vi "Run Panel VI.vi"(8 "error in (no error)":errorcluster, 11 "Panel in":refnum<class "Panel.lvclass">) -> (0 "error out":errorcluster, 3 "Panel out":refnum<class "Panel.lvclass">)   [LabVIEW 2020, in "OOPanel.lvlib" / "Panel.lvclass"]
uses:
  Panel.lvclass
  Panel.lvclass/Panel.ctl
  Visibility State.ctl
  <vilib>/Utility/error.llb/Error Cluster From Error Code.vi
  <vilib>/ErrorRing/Error Ring.xnode
  OOPanel.lvlib
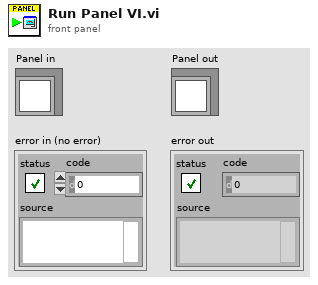
[diagram p1: front panel]
types:
  T1 = typedef "OOPanel.lvlib/Visibility State.ctl" = enum16{"Idle", "Closed", "Hidden", "Visible", "Subpanel", "Hidden Subpanel"}
  T2 = enum32{"invalid scope", "public", "private", "protected", "community"}
  T3 = enum32{"Invalid", "Standard", "Closed", "Hidden", "Minimized", "Maximized"}
  T4 = typedef "OOPanel.lvlib/Panel.lvclass/Ref Data.ctl" = cluster{"Panel Ref":refnum<vi>, "SubPanel":refnum<vi>, "Close":bool, "Running":bool, "State":T1}
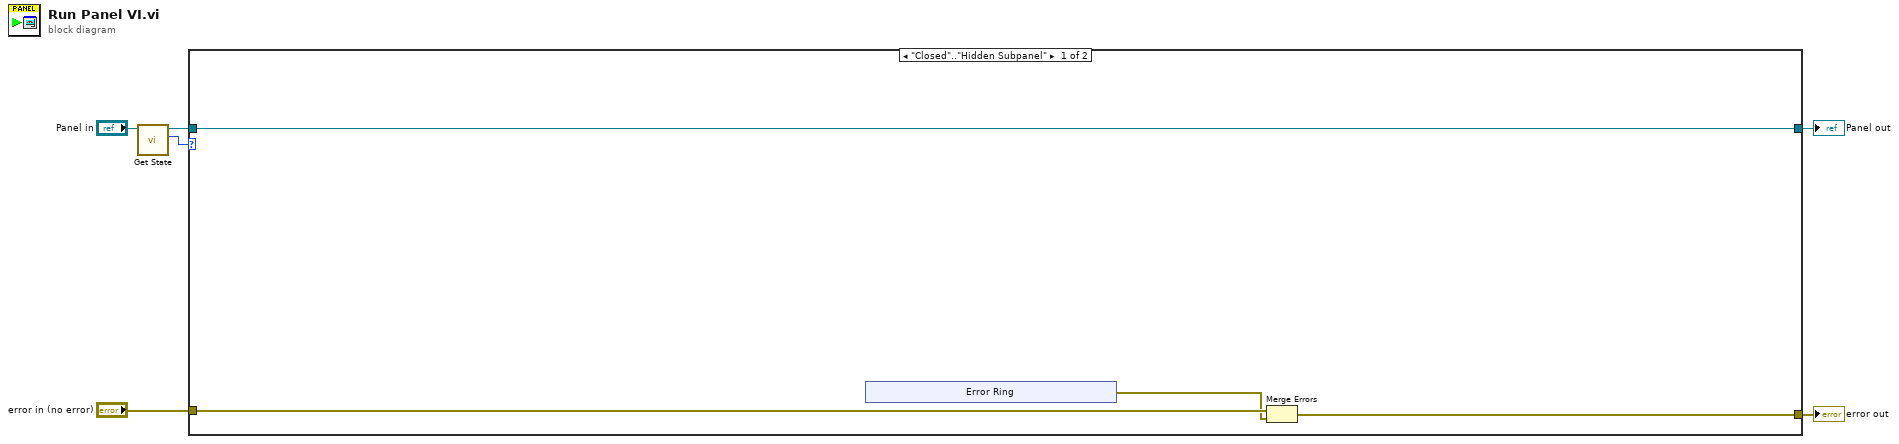
[diagram p0: block diagram]
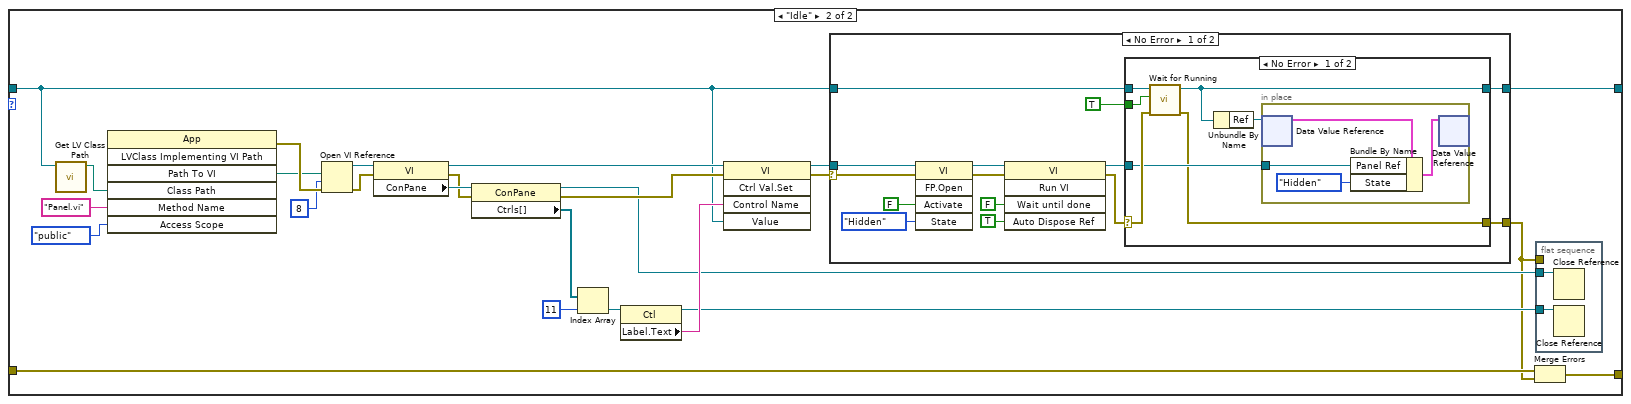
[diagram p2: hidden frame]
diagram:
  n1 = call "Get State.vi"("Panel in"="Panel in") -> ("State"=w1:T1, "Panel out"=w2:refnum<class "Panel.lvclass">)  [unwired: 8 in, 1 out]
  n2 = case shown="\"Closed\"..\"Hidden Subpanel\"" w1 {
    tunnel: "error in (no error)" -> [w9 w38]
    tunnel: [w10 w24] -> w5
    tunnel: [w7 w23] -> w4
    tunnel: w2 -> [w10 w18]
    frame "Closed".."Hidden Subpanel" {
      n3 = xnode "Error Ring"() -> ("error out"=w8:errorcluster)
      n4 = Merge Errors(w9, w8) -> (w7:errorcluster)
    }
    frame "Idle" {
      n5 = call <vilib>:"Get LV Class Path.vi"("object"=w18) -> ("class path"=w17:path)  [unwired: 9 in, 1 out]
      n6 = invoke class="App" method="LVClass Implementing VI Path"("Class Path"=w17, "Method Name"="Panel.vi", "Access Scope"=T2."public") -> (error out=w39:errorcluster, "Path To VI"=w16:path)  [unwired: 4 in, 5 out]
      n7 = Open VI Reference(vi path=w16, options=8, error in (no error)=w39) -> (vi reference=w37:refnum<vi>, error out=w36:errorcluster)  [unwired: 3 in]
      n8 = property class="VI"(reference=w37, error in=w36) -> (reference out=w32:refnum<vi>, error out=w30:errorcluster, "ConPane"=w35:refnum<vi>)
      n9 = property class="ConPane"(reference=w35, error in=w30) -> (reference out=w25:refnum<vi>, error out=w29:errorcluster, "Ctrls[]"=w34:refnum<vi>[])
      n10 = Index Array(array=w34, index=11) -> (element=w33:refnum<vi>)
      n11 = property class="Ctl"(reference=w33) -> (reference out=w26:refnum<vi>, "Label.Text"=w31:string)  [unwired: 1 in, 1 out]
      n12 = invoke class="VI" method="Ctrl Val.Set"(reference=w32, error in=w29, "Control Name"=w31, "Value"=w18) -> (reference out=w21:refnum<vi>, error out=w27:errorcluster)  [unwired: 1 in, 3 out]
      n13 = case shown="No Error" w27 {
        selector: w27 -> [w46 w69]
        tunnel: w21 -> [w47 _]
        tunnel: [w48 w69] -> w22
        tunnel: w18 -> [w52 w70]
        tunnel: [w51 w70] -> w24
        frame No Error {
          n14 = invoke class="VI" method="FP.Open"(reference=w47, error in=w46, "Activate"=FALSE ("Activate?"), "State"=T3."Hidden") -> (reference out=w43:refnum<vi>, error out=w42:errorcluster)  [unwired: 1 in, 3 out]
          n15 = invoke class="VI" method="Run VI"(reference=w43, error in=w42, "Wait until done"=FALSE ("Wait Until Done"), "Auto Dispose Ref"=TRUE ("Auto Dispose Reference")) -> (reference out=w53:refnum<vi>, error out=w49:errorcluster)  [unwired: 1 in, 3 out]
          n16 = case shown="No Error" w49 {
            selector: w49 -> [w58 w68]
            tunnel: w53 -> [w57 _]
            tunnel: w52 -> [w61 w67]
            tunnel: [w60 w67] -> w51
            tunnel: TRUE ("Running") -> [w59 _]
            tunnel: [w56 w68] -> w48
            frame No Error {
              n17 = call "Wait for Running.vi"("error in (no error)"=w58, "Running"=w59, "Panel in"=w61) -> ("error out"=w56:errorcluster, "Panel out"=w60:refnum<class "Panel.lvclass">)  [unwired: 7 in]
              n18 = Unbundle By Name(w60) -> ("Ref"=w62:refnum<data-value>)
              n19 = in-place {
                in-place-border: w57 -> [w63]
                n20 = in-place-dvr #1(w62) -> (w66:T4)  [unwired: 1 out]
                n21 = Bundle By Name(cluster=w66, "Panel Ref"=w63, "State"=Visibility_State."Hidden") -> (w65:T4)
                n22 = in-place-dvr #1(w65) -> ()  [unwired: 2 out]
              }
            }
            frame Error {
            }
          }
        }
        frame Error {
        }
      }
      n23 = Merge Errors(w38, w22) -> (w23:errorcluster)
      n24 = flat-sequence {
        tunnel: w26 -> [w41]
        tunnel: [w40] -> _
        tunnel: w25 -> [w40]
        tunnel: w22 -> [_]
        frame #0 {
          n25 = Close Reference(reference=w40) -> ()  [unwired: 1 in, 1 out]
          n26 = Close Reference(reference=w41) -> ()  [unwired: 1 in, 1 out]
        }
      }
    }
  }
  "error out" <- w4
  "Panel out" <- w5
